vi "CSM_Item_OnPopupMenu.vi"(11 "Object":T1) -> ()   [LabVIEW 2017]
uses:
  <resource>/Framework/Providers/API/ItemRef.ctl
  <resource>/Framework/Providers/API/mxLvMenuItem.ctl
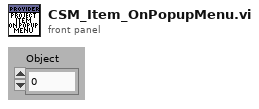
[diagram p1: front panel]
types:
  T1 = typedef "ItemRef.ctl" = u64
  T2 = typedef "mxLvMenuItem.ctl" = cluster{"Menu Name":string, "Description":string, "Icon File Name":path, "Menu Tag":string, "Enabled":bool, "Checked":bool, "Separator":bool, "Batchable":bool, "Weight":i32, "Batch Mode (Ignored if Not Batchable)":enum32{"Show If All Items Support Command", "Show If Any Items Support Command"}, "Menu Location":enum32{"<None>", "Project", "Project / Build Specifications", "Tools", "Tools / Source Control", "Tools / Real-Time Module", "Help"}, "Exclude From Getting Started Window Menu":bool}
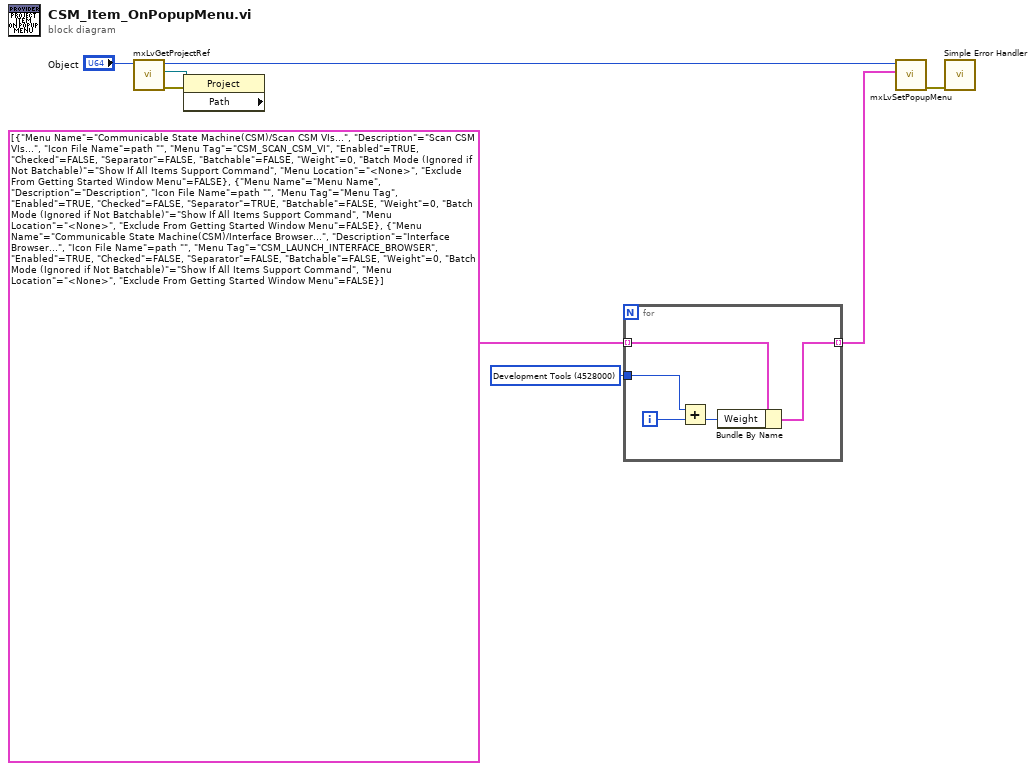
[diagram p0: block diagram]
diagram:
  w1 = u32 4528000 items=["DEV_Env"=4520000, "<2>"=1, "<3>"=2, "SystemProviders"=4523000, "<5>"=4, "<6>"=5, "ToolProviders"=4527000, "Development Tools"=4528000, "Git"=4529000] ("Ring")
  n1 = call <resource>:"mxLvGetProjectRef.vi"("Item"="Object") -> ("error out"=w6:errorcluster, "Project Refnum"=w5:refnum<vi>, "Item"=w4:T1)  [unwired: 8 in]
  n2 = property class="Project" props=["Path"](reference=w5, error in=w6) -> ()  [unwired: 3 out]
  n3 = for {
    tunnel: T2[] [{"Menu Name"="Communicable State Machine(CSM)/Scan CSM VIs...", "Description"="Scan CSM VIs...", "Icon File Name"=path "", "Menu Tag"="CSM_SCAN_CSM_VI", "Enabled"=TRUE, "Checked"=FALSE, "Separator"=FALSE, "Batchable"=FALSE, "Weight"=0, "Batch Mode (Ignored if Not Batchable)"=enum."Show If All Items Support Command", "Menu Location"=enum."<None>", "Exclude From Getting Started Window Menu"=FALSE}, {"Menu Name"="Menu Name", "Description"="Description", "Icon File Name"=path "", "Menu Tag"="Menu Tag", "Enabled"=TRUE, "Checked"=FALSE, "Separator"=TRUE, "Batchable"=FALSE, "Weight"=0, "Batch Mode (Ignored if Not Batchable)"=enum."Show If All Items Support Command", "Menu Location"=enum."<None>", "Exclude From Getting Started Window Menu"=FALSE}, {"Menu Name"="Communicable State Machine(CSM)/Interface Browser...", "Description"="Interface Browser...", "Icon File Name"=path "", "Menu Tag"="CSM_LAUNCH_INTERFACE_BROWSER", "Enabled"=TRUE, "Checked"=FALSE, "Separator"=FALSE, "Batchable"=FALSE, "Weight"=0, "Batch Mode (Ignored if Not Batchable)"=enum."Show If All Items Support Command", "Menu Location"=enum."<None>", "Exclude From Getting Started Window Menu"=FALSE}] ("Array") -> [w13] mode=indexing
    tunnel: [w12] -> w2 mode=indexing
    tunnel: w1 -> [w9]
    i -> [w11]
    n4 = Add(x=w9, y=w11) -> (x+y=w10:u32)
    n5 = Bundle By Name(cluster=w13, "Weight"=w10) -> (w12:T2)
  }
  n6 = call <resource>:"mxLvSetPopupMenu.vi"("Popup Menu Items"=w2, "Item"=w4) -> ("error out"=w8:errorcluster)  [unwired: 8 in, 1 out]
  n7 = call <vilib>:"Simple Error Handler.vi"("error in (no error)"=w8) -> ()  [unwired: 4 in, 5 out]
